vi "Logging Cascade Pos.vi"(11 "Sensor Position":dbl) -> ()   [LabVIEW 2027]
uses:
  <vilib>/MRC/MrcLib.lvlib
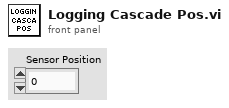
[diagram p1: front panel]
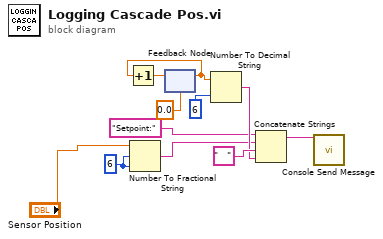
[diagram p0: block diagram]
diagram:
  w10 = i16 6 ("width (-)")
  n1 = Number To Fractional String(number="Sensor Position", width (-)=w10, precision (6)=w10) -> (F-format string=w3:string)  [unwired: 1 in]
  n2 = feedback #1(0.0) -> (w11:dbl)
  n3 = Increment(x=w11) -> (x+1=w6:dbl)
  n4 = feedback-in #1(w6) -> ()
  n5 = Number To Decimal String(number=w11, width (-)=i16 6) -> (decimal integer string=w8:string)
  n6 = Concatenate Strings("Setpoint:" ("string"), w3, "   " ("string"), w8) -> (w1:string)
  n7 = call <vilib>:"Console Send Message.vi"("Message"=w1) -> ()  [unwired: 14 in, 1 out]
